vi "RDC-permittivity_collection.vi"(7 "basic data(open, short, water)":T2[](array[typedef]), 8 "Perm calc type":T1, 11 "Common Format":T2) -> (3 "Common Format 2":T2)   [LabVIEW 2020, in "RDC-Reflection_Data_Computation.lvlib"]
doc: "Computes the permittivity of a Common Format cluster with the method chosen in Perm calc type (Basic, Capacative, Advance or Bilinear), using the basic data."
uses:
  RDC-Reflection_Data_Computation.lvlib
  Reflector/RFH-common_data_format.ctl
  RDC-perm_calc_type.ctl
  Reflector/RFH-Reflection_File_Handler.lvlib
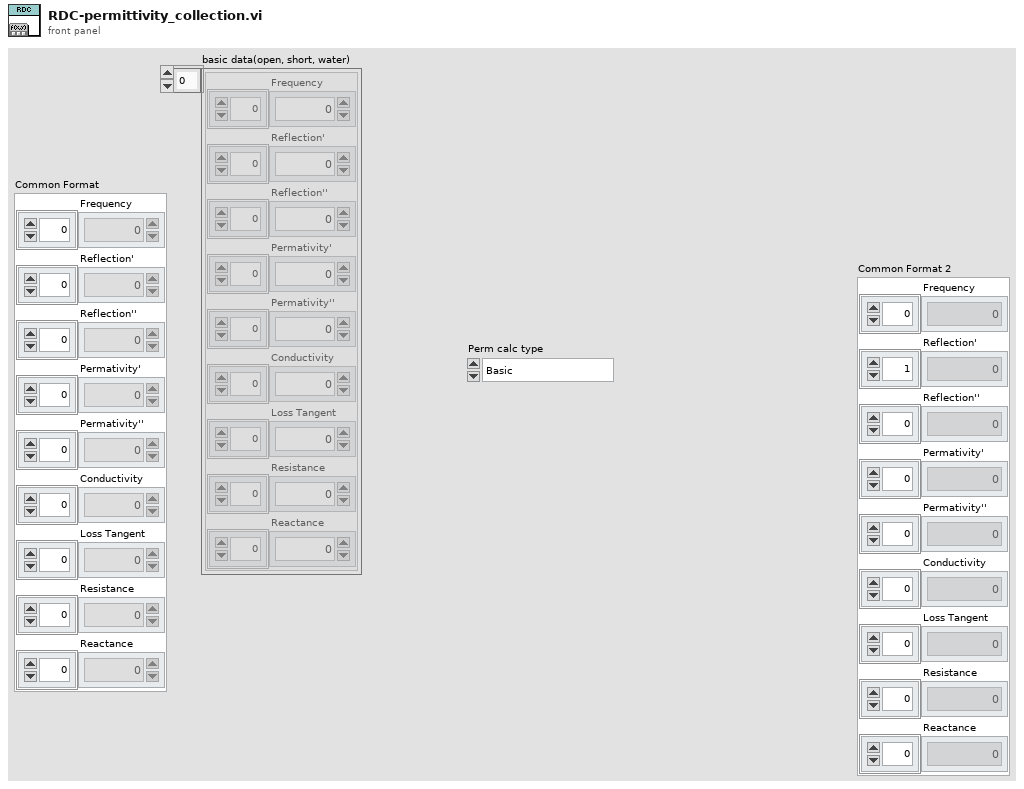
[diagram p1: front panel]
types:
  T1 = typedef "RDC-Reflection_Data_Computation.lvlib/RDC-perm_calc_type.ctl" = enum16{"Basic", "Capacative", "Advance", "Bilinear", "Size"}
  T2 = typedef "RFH-Reflection_File_Handler.lvlib/RFH-common_data_format.ctl" = cluster{"Frequency":dbl[], "Reflection'":dbl[], "Reflection''":dbl[], "Permativity'":dbl[], "Permativity''":dbl[], "Conductivity":dbl[], "Loss Tangent":dbl[], "Resistance":dbl[], "Reactance":dbl[]}
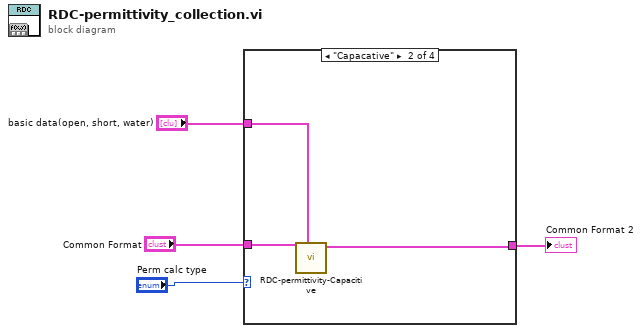
[diagram p0: block diagram]
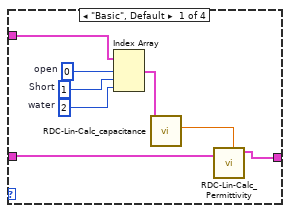
[diagram p2: hidden frame]
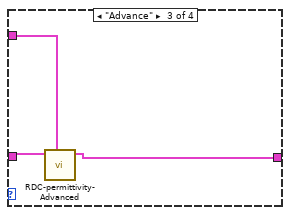
[diagram p3: hidden frame]
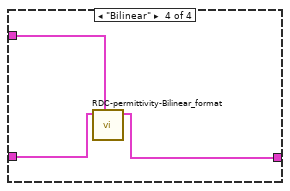
[diagram p4: hidden frame]
diagram:
  n1 = case shown="\"Capacative\"" "Perm calc type" {
    tunnel: "Common Format" -> [w11 w14 w18 w20]
    tunnel: [w10 w13 w16 w19] -> w3
    tunnel: "basic data(open, short, water)" -> [w9 w15 w17 w21]
    frame "Basic", Default {
      w6 = 2  # water
      w7 = 1  # Short
      w8 = 0  # open
      n2 = Index Array(array=w9, index #1=w8, index #2=w7, index #3=w6) -> (element #1=w5:T2)  [unwired: 2 out]
      n3 = call "RDC-Lin-Calc_capacitance.vi"("Open Probe reading"=w5) -> ("C0"=w12:dbl)  [unwired: 9 in, 1 out]
      n4 = call "RDC-Lin-Calc_Permittivity.vi"("C0"=w12, "input cluster"=w11) -> ("Output cluster"=w10:T2)  [unwired: 9 in]
    }
    frame "Capacative" {
      n5 = call "RDC-permittivity-Capacitive.vi"("basic data(open, short, water)"=w15, "Common Format"=w14) -> ("Common Format 2"=w13:T2)  [unwired: 9 in]
    }
    frame "Advance" {
      n6 = call "RDC-permittivity-Advanced.vi"("basic data(open, short, water)"=w17, "Common Format"=w18) -> ("Common Format out"=w16:T2)  [unwired: 9 in]
    }
    frame "Bilinear" {
      n7 = call "RDC-permittivity-Bilinear_format.vi"("basic data(open, short, water)"=w21, "Common Format"=w20) -> ("Common Format out"=w19:T2)  [unwired: 9 in]
    }
  }
  "Common Format 2" <- w3
